vi "SA set DisplayLine.vi"(8 "error in (no error)":errorcluster caption="에러 입력(에러 없음)", 10 "Amplitude":dbl, 11 "Instrument Manager 입력":refnum<class "Instrument Manager.lvclass">) -> (0 "error out":errorcluster caption="에러 출력", 3 "Instrument Manager 출력":refnum<class "Instrument Manager.lvclass">)   [LabVIEW 2023, in "Instrument Manager.lvclass"]
uses:
  Instrument Manager.lvclass
  Instrument Manager.lvclass/Instrument Manager.ctl
  Module/Spectrum Analyzer/Interface_Spectrum/Interface_Spectrum.lvclass
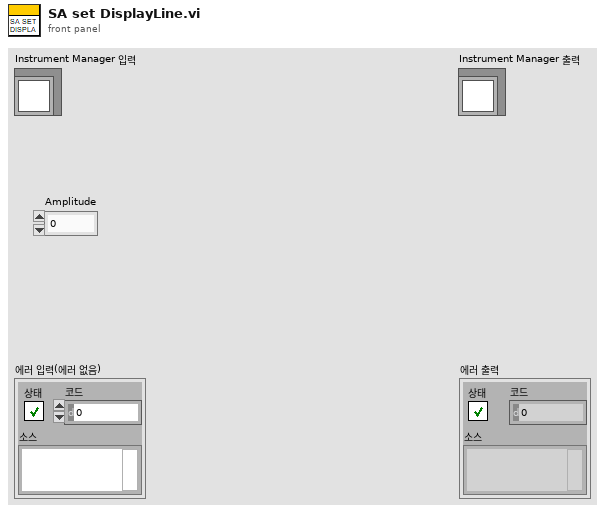
[diagram p1: front panel]
types:
  T1 = cluster{"Anritsu Call Box":refnum<class "Anritsu Call Box.lvclass">, "Spectrum Analyzer":refnum<class "Interface_Spectrum.lvclass">, "RF Switch Box":refnum<class "RF Filter Box.lvclass">, "Turn Table":refnum<class "Interface - Turn Table.lvclass">, "Mast":refnum<class "Interface - Mast.lvclass">, "3D Controller":refnum<class "Interface_3D Controller.lvclass">}
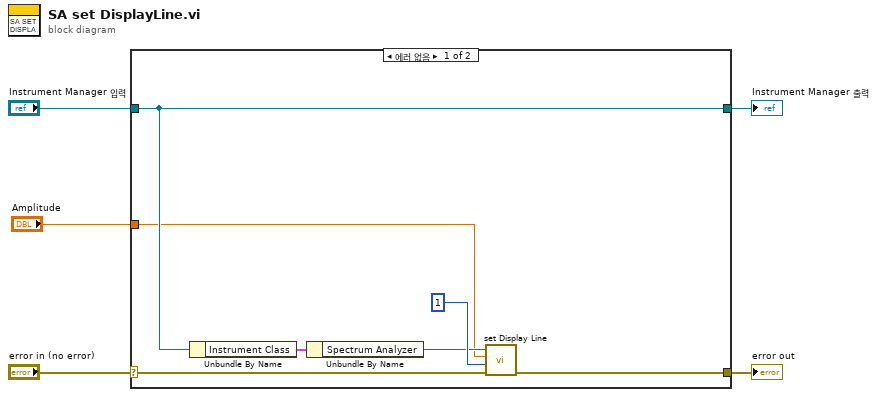
[diagram p0: block diagram]
diagram:
  n1 = case shown="에러 없음" "error in (no error)" {
    selector: "error in (no error)" -> [w9 w14]
    tunnel: [w8 w14] -> w4
    tunnel: [w12 w13] -> w2
    tunnel: "Instrument Manager 입력" -> [w12 w13]
    tunnel: "Amplitude" -> [w6 _]
    frame No Error {
      n2 = Unbundle By Name(w12) -> ("Instrument Class"=w11:T1)
      n3 = Unbundle By Name(w11) -> ("Spectrum Analyzer"=w7:refnum<class "Interface_Spectrum.lvclass">)
      n4 = call-dynamic "set Display Line.vi"("error in (no error)"=w9, "Line Index"=1, "Amplitude"=w6, "Interface_Spectrum in"=w7) -> ("error out"=w8:errorcluster)  [unwired: 6 in, 1 out]
    }
    frame Error {
    }
  }
  "error out" <- w4
  "Instrument Manager 출력" <- w2
